vi "Rx Update Rate Timer FGV.vi"(8 "error in":errorcluster, 10 "Desired Updated Rate (mSec)":u32 caption="Tick Count(mSec)", 11 "Operation":enum16{"Reset", "Check"}(ring)) -> (0 "error out":errorcluster, 2 "Elapsed Time (mS)":u32, 3 "Ready?":bool)   [LabVIEW 2015, in "Two Way Event Recorder Custom Device.lvlib"]
uses:
  Two Way Event Recorder Custom Device.lvlib
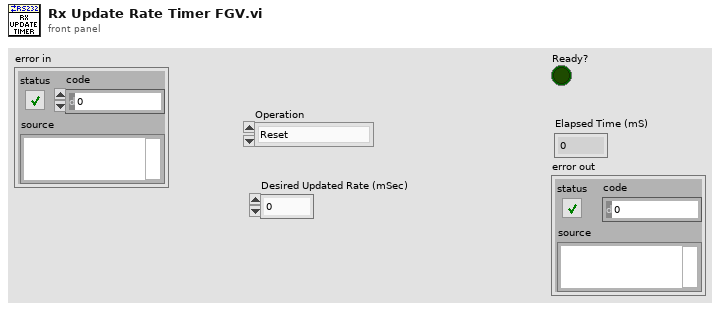
[diagram p1: front panel]
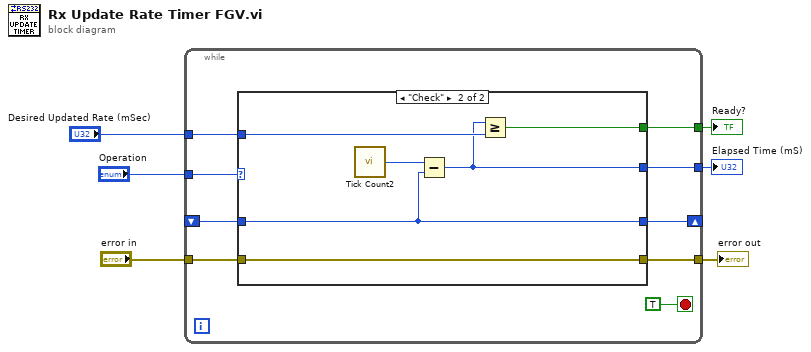
[diagram p0: block diagram]
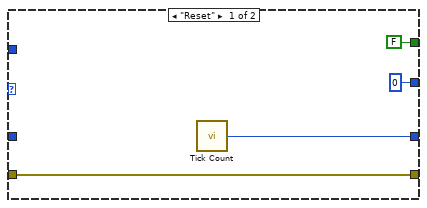
[diagram p2: hidden frame]
diagram:
  n1 = while {
    tunnel: "Operation" -> [w14]
    shift-right: [w13] -> _
    shift-left: _ -> [w12]
    tunnel: "Desired Updated Rate (mSec)" -> [w11]
    tunnel: [w10] -> w5
    tunnel: [w9] -> w4
    tunnel: "error in" -> [w8]
    tunnel: [w7] -> w1
    stop <- TRUE stop-if-true
    n2 = case shown="\"Check\"" w14 {
      tunnel: [w19 w24] -> w13
      tunnel: w12 -> [_ w24]
      tunnel: w11 -> [_ w23]
      tunnel: [FALSE w22] -> w10
      tunnel: [u32 0 w21] -> w9
      tunnel: [w16 w20] -> w7
      tunnel: w8 -> [w16 w20]
      frame "Reset" {
        n3 = call "Tick Count"() -> ("Tick Count(uSec)"=w19:u32)
      }
      frame "Check" {
        n4 = call "Tick Count2"() -> ("Tick Count(mSec)"=w25:u32)
        n5 = Subtract(x=w25, y=w24) -> (x-y=w21:u32)
        n6 = Greater Or Equal?(x=w21, y=w23) -> (x >= y?=w22:bool)
      }
    }
  }
  "Ready?" <- w5
  "Elapsed Time (mS)" <- w4
  "error out" <- w1
